vi "subXMLGetDestinationDir.vi"(9 "Project path":path, 10 "TargetName":string, 11 "Refnum in":refnum<k20>) -> (1 "Name":string, 3 "Path":path)   [LabVIEW 2019, in "SolutionBuilder.lvlib" / "SolutionBuilder.lvclass"]
uses:
  SolutionBuilder.lvclass
  <vilib>/xml/NI_XML.lvlib
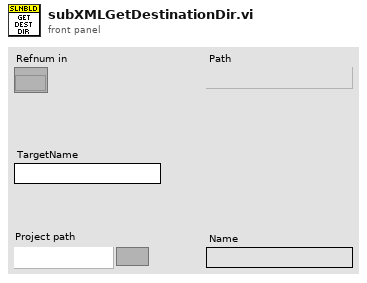
[diagram p1: front panel]
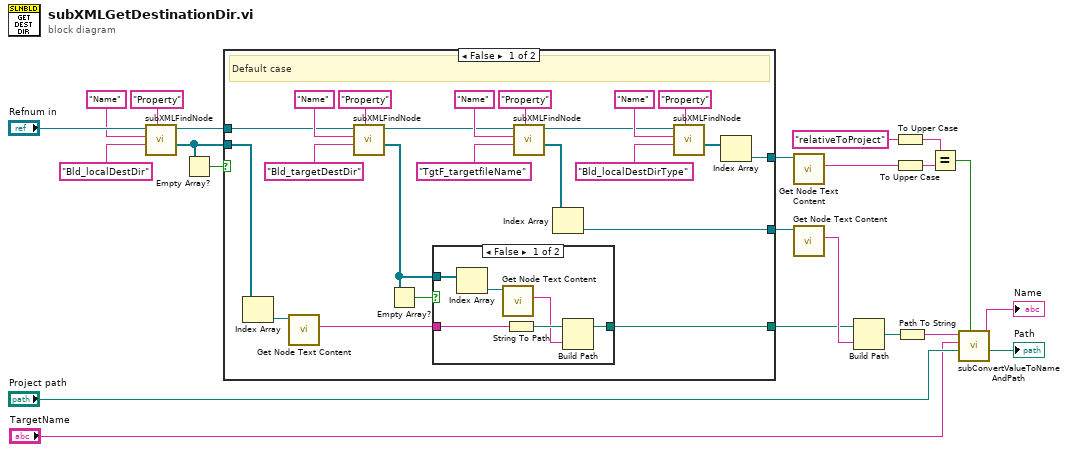
[diagram p0: block diagram]
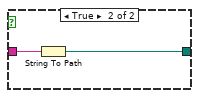
[diagram p2: hidden frame]
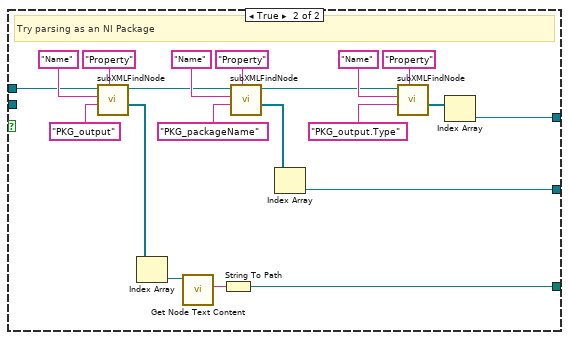
[diagram p3: hidden frame]
diagram:
  n1 = call "subXMLFindNode.vi"("Node name"="Property", "Property value"="Bld_localDestDir", "Property name"="Name", "Refnum in"="Refnum in") -> ("Nodes"=w8:refnum<k20>[], "Refnum"=w11:refnum<k20>)  [unwired: 6 in]
  n2 = Empty Array?(array=w8) -> (empty?=w7:bool)
  n3 = case shown="False" w7 {
    tunnel: w8 -> [w43 _]
    tunnel: [w39 w59] -> w15
    tunnel: w11 -> [w34 w69]
    tunnel: [w29 w65] -> w10
    tunnel: [w23 w53] -> w6
    frame False {
      # "Default case"
      n4 = Index Array(array=w43) -> (element=w44:refnum<k20>)  [unwired: 1 in]
      n5 = call <vilib>:"Get Node Text Content.vi"("node in"=w44) -> ("node text"=w30:string)  [unwired: 8 in, 2 out]
      n6 = call "subXMLFindNode.vi"("Node name"="Property", "Property value"="Bld_targetDestDir", "Property name"="Name", "Refnum in"=w34) -> ("Nodes"=w32:refnum<k20>[], "Refnum"=w33:refnum<k20>)  [unwired: 6 in]
      n7 = Empty Array?(array=w32) -> (empty?=w31:bool)
      n8 = case shown="False" w31 {
        tunnel: w32 -> [w49 _]
        tunnel: w30 -> [w47 w52]
        tunnel: [w45 w51] -> w29
        frame False {
          n9 = Index Array(array=w49) -> (element=w50:refnum<k20>)  [unwired: 1 in]
          n10 = call <vilib>:"Get Node Text Content.vi"("node in"=w50) -> ("node text"=w46:string)  [unwired: 8 in, 2 out]
          n11 = String To Path(string=w47) -> (path=w48:path)
          n12 = Build Path(base path=w48, name or relative path=w46) -> (appended path=w45:path)
        }
        frame True {
          n13 = String To Path(string=w52) -> (path=w51:path)
        }
      }
      n14 = call "subXMLFindNode.vi"("Node name"="Property", "Property value"="TgtF_targetfileName", "Property name"="Name", "Refnum in"=w33) -> ("Nodes"=w40:refnum<k20>[], "Refnum"=w24:refnum<k20>)  [unwired: 6 in]
      n15 = Index Array(array=w40) -> (element=w39:refnum<k20>)  [unwired: 1 in]
      n16 = call "subXMLFindNode.vi"("Node name"="Property", "Property value"="Bld_localDestDirType", "Property name"="Name", "Refnum in"=w24) -> ("Nodes"=w27:refnum<k20>[])  [unwired: 6 in, 1 out]
      n17 = Index Array(array=w27) -> (element=w23:refnum<k20>)  [unwired: 1 in]
    }
    frame True {
      # "Try parsing as an NI Package"
      n18 = call "subXMLFindNode.vi"("Node name"="Property", "Property value"="PKG_output", "Property name"="Name", "Refnum in"=w69) -> ("Nodes"=w67:refnum<k20>[], "Refnum"=w61:refnum<k20>)  [unwired: 6 in]
      n19 = Index Array(array=w67) -> (element=w68:refnum<k20>)  [unwired: 1 in]
      n20 = call <vilib>:"Get Node Text Content.vi"("node in"=w68) -> ("node text"=w66:string)  [unwired: 8 in, 2 out]
      n21 = String To Path(string=w66) -> (path=w65:path)
      n22 = call "subXMLFindNode.vi"("Node name"="Property", "Property value"="PKG_packageName", "Property name"="Name", "Refnum in"=w61) -> ("Nodes"=w60:refnum<k20>[], "Refnum"=w54:refnum<k20>)  [unwired: 6 in]
      n23 = Index Array(array=w60) -> (element=w59:refnum<k20>)  [unwired: 1 in]
      n24 = call "subXMLFindNode.vi"("Node name"="Property", "Property value"="PKG_output.Type", "Property name"="Name", "Refnum in"=w54) -> ("Nodes"=w57:refnum<k20>[])  [unwired: 6 in, 1 out]
      n25 = Index Array(array=w57) -> (element=w53:refnum<k20>)  [unwired: 1 in]
    }
  }
  n26 = call <vilib>:"Get Node Text Content.vi"("node in"=w6) -> ("node text"=w4:string)  [unwired: 8 in, 2 out]
  n27 = call <vilib>:"Get Node Text Content.vi"("node in"=w15) -> ("node text"=w14:string)  [unwired: 8 in, 2 out]
  n28 = Build Path(base path=w10, name or relative path=w14) -> (appended path=w13:path)
  n29 = To Upper Case(1:"relativeToProject" ("node text")) -> (0:w3:string)
  n30 = To Upper Case(1:w4) -> (0:w2:string)
  n31 = Path To String(path=w13) -> (string=w12:string)
  n32 = Equal?(x=w3, y=w2) -> (x = y?=w1:bool)
  n33 = call "subConvertValueToNameAndPath.vi"("RelativeToProject"=w1, "Project path"="Project path", "TargetName"="TargetName", "Value"=w12) -> ("Path"=→"Path":path, "Name"=→"Name":string)  [unwired: 6 in]
